vi "Read I32.vi"(7 "key":string, 8 "error in (no error)":errorcluster, 9 "default value":i32, 11 "Configuration File In":refnum<class "Configuration File.lvclass">) -> (0 "error out":errorcluster, 1 "value":i32, 3 "Configuration File Out":refnum<class "Configuration File.lvclass">)   [LabVIEW 2020, in "Configuration File.lvclass"]
doc: "High-level function for reading configuration file data from process class. If the specified key is not present, it is added with the configured default value."
uses:
  Configuration File.lvclass
  C:/Git/astemes-triarc-framework/source/Framework/Configuration/Configuration.lvclass
  Base/Base.lvclass/Base.ctl
  Base/Public/Read Base Name.vi
  Private/Read Config File Ref.vi
  Configuration/Protected/Get Config Ref.vi
  <vilib>/Utility/error.llb/Clear Errors.vi
  Process/Public/Read Name.vi
  <vilib>/Utility/config.llb/Not A Config Data Refnum.vi
  <vilib>/Utility/config.llb/Read Key (I32).vi
  Process/Process.lvclass
  Base/Base.lvclass
  <vilib>/Utility/config.llb/NI_LVConfig.lvlib
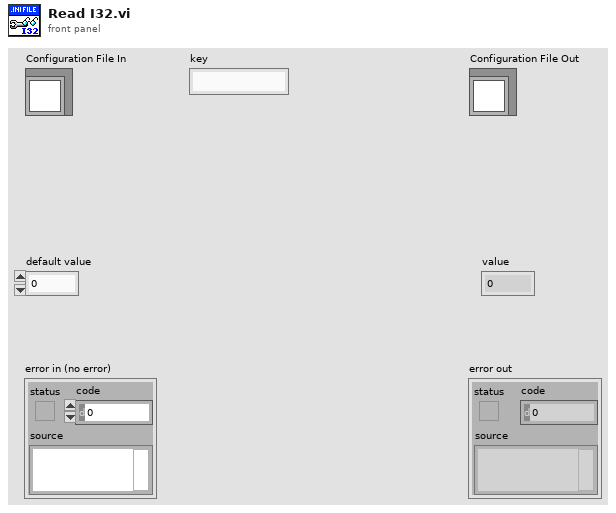
[diagram p1: front panel]
types:
  T1 = typedef "NI_LVConfig.lvlib/Config Data RefNum.ctl" = refnum<k1>
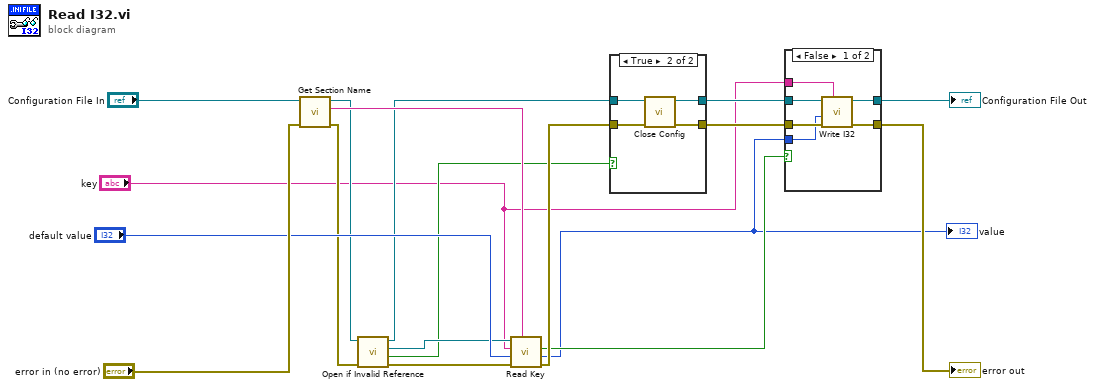
[diagram p0: block diagram]
diagram:
  n1 = call "Get Section Name.vi"("error in (no error)"="error in (no error)", "Configuration File In"="Configuration File In") -> ("error out"=w12:errorcluster, "Section Name"=w15:string, "Configuration File Out"=w14:refnum<class "Configuration File.lvclass">)  [unwired: 7 in]
  n2 = call "Open if Invalid Reference.vi"("error in (no error)"=w12, "Configuration File In"=w14) -> ("error out"=w11:errorcluster, "File opened?"=w3:bool, "refnum out"=w10:T1, "Configuration File Out"=w13:refnum<class "Configuration File.lvclass">)  [unwired: 6 in]
  n3 = call-poly <vilib>:"Read Key.vi"("section"=w15, "error in (no error)"=w11, "default value"="default value", "key"="key", "refnum"=w10) -> ("error out"=w7:errorcluster, "value"=w2:i32, "found?"=w4:bool)  [unwired: 3 in, 1 out]
  "value" <- w2
  n4 = case shown="True" w3 {
    tunnel: w13 -> [w20 w24]
    tunnel: [w20 w23] -> w9
    tunnel: w7 -> [w19 w22]
    tunnel: [w19 w21] -> w6
    frame False {
    }
    frame True {
      n5 = call-dynamic "Close Config.vi"("error in (no error)"=w22, "Configuration File File In"=w24) -> ("error out"=w21:errorcluster, "Configuration File File Out"=w23:refnum<class "Configuration File.lvclass">)  [unwired: 8 in]
    }
  }
  n6 = case shown="False" w4 {
    tunnel: w9 -> [w30 w31]
    tunnel: [w29 w31] -> w8
    tunnel: w6 -> [w28 w32]
    tunnel: [w27 w32] -> w5
    tunnel: w2 -> [w26 _]
    tunnel: "key" -> [w25 _]
    frame False {
      n7 = call-dynamic "Write I32.vi"("key"=w25, "error in (no error)"=w28, "Value"=w26, "Configuration File In"=w30) -> ("error out"=w27:errorcluster, "Configuration File Out"=w29:refnum<class "Configuration File.lvclass">)  [unwired: 6 in]
    }
    frame True {
    }
  }
  "error out" <- w5
  "Configuration File Out" <- w8
